vi "Add To Library Files.vi"() -> (15 "error out":errorcluster)   [LabVIEW 2020]
doc: "Dev helper: like Add To Library Main2.vi but reads item paths and caller paths from text files (one path per line). In THIS application instance (no project): opens the library, adds every item with AddItem, opens a reference to each caller (so they relink), saves the modified library members (Save All This Library, only modified) and closes everything."
uses:
  <vilib>/Utility/EditLVLibs/Edit LVLibs.lvlib
panel:
  out "open code min":i32
  out "open code max":i32
  out "add code min":i32
  out "add code max":i32
  out "items added":i32
  in  "callers file":path
  in  "items file":path
  in  "library path":path
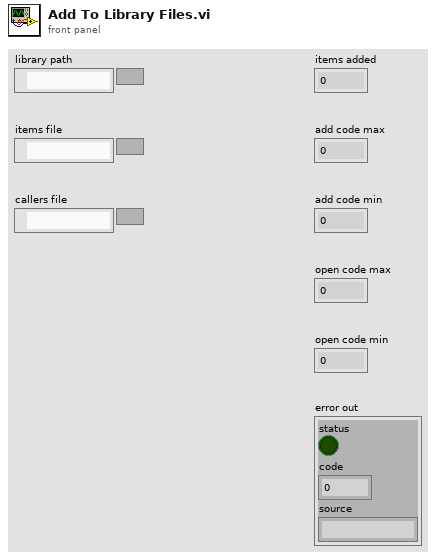
[diagram p1: front panel]
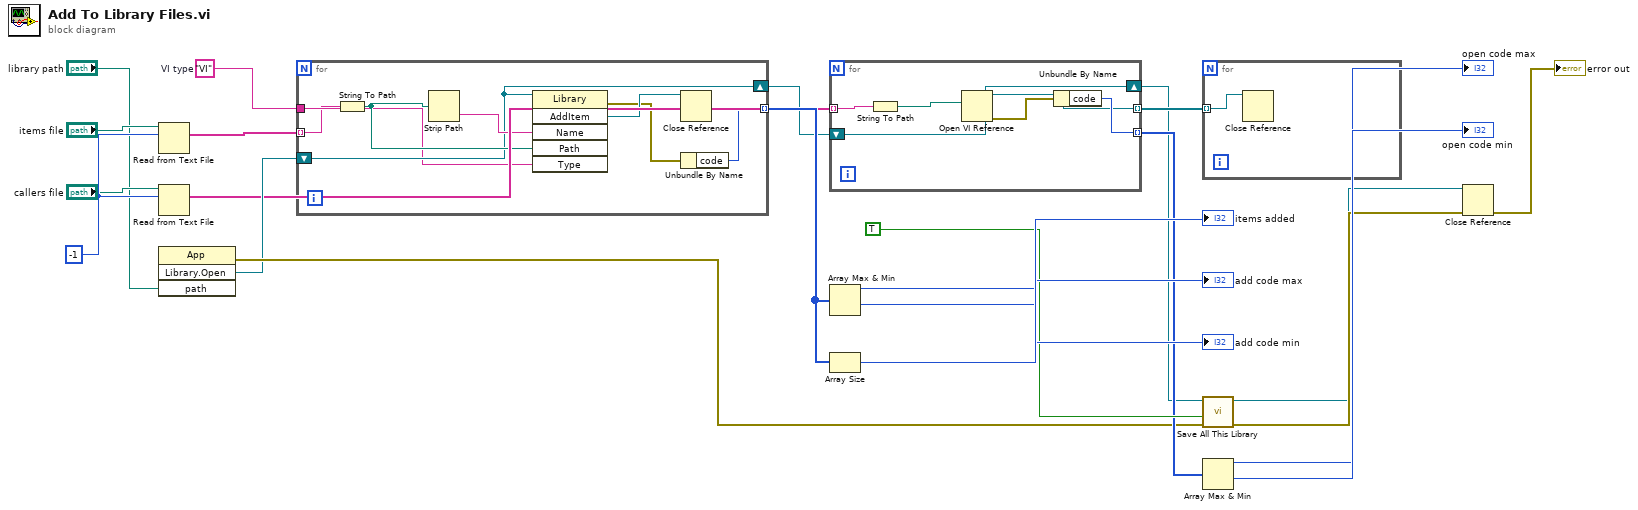
[diagram p0: block diagram]
diagram:
  w7 = "VI"  # VI type
  w4 = -1
  n1 = Read from Text File(file (use dialog)="items file", count=w4) -> (text=w5:string[])  [unwired: 2 in, 3 out]
  n2 = Read from Text File(file (use dialog)="callers file", count=w4) -> (text=w6:string[])  [unwired: 2 in, 3 out]
  n3 = invoke class="App" method="Library.Open"("path"="library path") -> (error out=w9:errorcluster, "Open Library"=w8:refnum<vi>)  [unwired: 3 in, 2 out]
  n4 = for {
    tunnel: w7 -> [w25]
    tunnel: w5 -> [w24] mode=indexing
    shift-right: [w26] -> w10
    shift-left: w8 -> [w26]
    tunnel: [w31] -> w11 mode=indexing
    n5 = String To Path(string=w24) -> (path=w27:path)
    n6 = Strip Path(path=w27) -> (name=w28:string)  [unwired: 1 out]
    n7 = invoke class="Library" method="AddItem"(reference=w26, "Name"=w28, "Path"=w27, "Type"=w25) -> (error out=w29:errorcluster, "AddItem"=w30:refnum<vi>)  [unwired: 2 in, 4 out]
    n8 = Close Reference(reference=w30) -> ()  [unwired: 1 in, 1 out]
    n9 = Unbundle By Name(w29) -> ("code"=w31:i32)
  }
  n10 = for {
    tunnel: w6 -> [w32] mode=indexing
    shift-right: [w33] -> w12
    shift-left: w10 -> [w33]
    tunnel: [w35] -> w13 mode=indexing
    tunnel: [w37] -> w14 mode=indexing
    n11 = String To Path(string=w32) -> (path=w34:path)
    n12 = Open VI Reference(vi path=w34) -> (vi reference=w35:refnum<vi>, error out=w36:errorcluster)  [unwired: 5 in]
    n13 = Unbundle By Name(w36) -> ("code"=w37:i32)
  }
  n14 = Array Max & Min(array=w11) -> (max value=→"add code max":i32, min value=→"add code min":i32)  [unwired: 2 out]
  n15 = Array Size(array=w11) -> (size(s)=→"items added":i32)
  n16 = for {
    tunnel: w13 -> [w38] mode=indexing
    n17 = Close Reference(reference=w38) -> ()  [unwired: 1 in, 1 out]
  }
  n18 = call <vilib>:"Save All This Library.vi"("error in (no error)"=w9, "Save Only Modified VIs and Libraries? (F)"=TRUE, "Library in"=w12) -> ("error out"=w17:errorcluster, "Library out"=w16:refnum<vi>)  [unwired: 7 in]
  n19 = Array Max & Min(array=w14) -> (max value=→"open code max":i32, min value=→"open code min":i32)  [unwired: 2 out]
  n20 = Close Reference(reference=w16, error in (no error)=w17) -> (error out=→"error out":errorcluster)
